vi "Subtract OutputOffset from Sweep Config.vi"(8 "error in (no error)":errorcluster, 11 "Instrument.DAQ":refnum<class "Instrument.DAQ.lvclass">) -> (0 "error out":errorcluster, 3 "Instrument.DAQ out":refnum<class "Instrument.DAQ.lvclass">)   [LabVIEW 2019, in "Instrument.Lockin.lvlib" / "Instrument.DAQ.lvclass"]
uses:
  Instrument.DAQ.lvclass
  Instrument.DAQ.lvclass/Instrument.DAQ.ctl
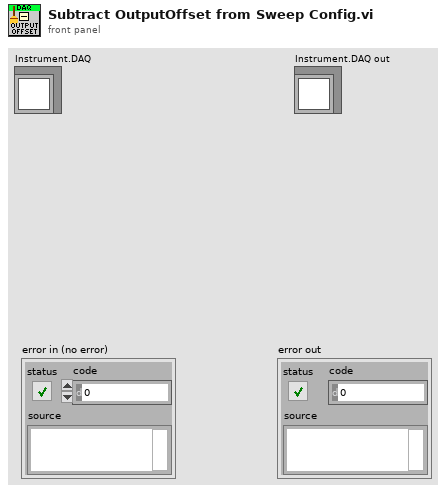
[diagram p1: front panel]
types:
  T1 = typedef "Instrument.Lockin.lvlib/Instrument.DAQ.lvclass/Sweep.Channel--Cluster--Array.ctl" = T2[]
  T2 = typedef "Instrument.Lockin.lvlib/Instrument.DAQ.lvclass/Sweep.Channel--Cluster.ctl" = cluster{"Enable?":bool, "Channel":i32, "Start":dbl, "End":dbl, "Pattern":T3, "Table":dbl[]}
  T3 = typedef "Instrument.Lockin.lvlib/Instrument.DAQ.lvclass/Sweep.Pattern--Enum.ctl" = enum16{"Ramp /", "Ramp /\\", "Smooth Ramp _/", "Smooth Ramp _/\\_", "Table"}
  T4 = typedef "Instrument.Lockin.lvlib/Instrument.DAQ.lvclass/Channel.Offset--Cluster--Array.ctl" = T5[]
  T5 = typedef "Instrument.Lockin.lvlib/Instrument.DAQ.lvclass/Channel.Offset--Cluster.ctl" = cluster{"Channel":string, "Offset":dbl}
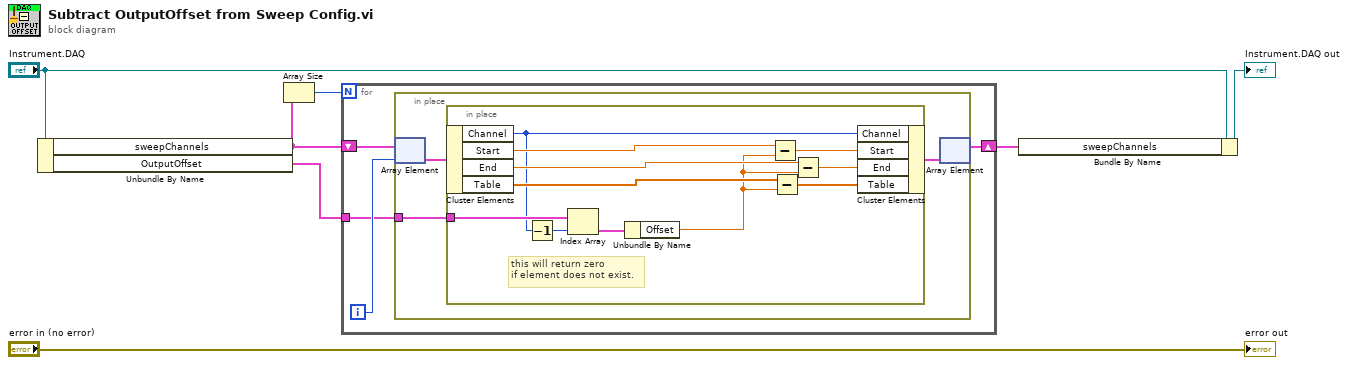
[diagram p0: block diagram]
diagram:
  n1 = Unbundle By Name("Instrument.DAQ") -> ("sweepChannels"=w5:T1, "OutputOffset"=w1:T4)
  n2 = Array Size(array=w5) -> (size(s)=w6:i32)
  n3 = for {
    N: w6 -> [_]
    tunnel: w1 -> [w8]
    shift-right: [w11] -> w2
    shift-left: w5 -> [w9]
    i -> [w10]
    n4 = in-place {
      in-place-border: w8 -> [w12]
      n5 = in-place-array #1(w9, w10) -> (w13:T2)
      n6 = in-place {
        in-place-border: w12 -> [w18]
        # "this will return zero\nif element does not exist."
        n7 = in-place-cluster #2(w13) -> ("Channel"=w16:i32, "Start"=w25:dbl, "End"=w23:dbl, "Table"=w21:dbl[])
        n8 = Decrement(x=w16) -> (x-1=w17:i32)
        n9 = Index Array(array=w18, index=w17) -> (element=w19:T5)
        n10 = Unbundle By Name(w19) -> ("Offset"=w15:dbl)
        n11 = Subtract(x=w25, y=w15) -> (x-y=w24:dbl)
        n12 = Subtract(x=w21, y=w15) -> (x-y=w20:dbl[])
        n13 = Subtract(x=w23, y=w15) -> (x-y=w22:dbl)
        n14 = in-place-cluster #2("Channel"=w16, "Start"=w24, "End"=w22, "Table"=w20) -> (w14:T2)
      }
      n15 = in-place-array #1(w14) -> (w11:T1)  [unwired: 1 out]
    }
  }
  n16 = Bundle By Name(cluster="Instrument.DAQ", "sweepChannels"=w2) -> (→"Instrument.DAQ out":refnum<class "Instrument.DAQ.lvclass">)
  "error out" <- "error in (no error)"
